vi "CIVI Basic Control Example.vi"() -> ()   [LabVIEW 2026]
panel:
  in  "Frequency Setpoint (Hz)":i32=774000
  out "SCPI Error Code":i32
  in  "Mode Setpint":string="AM"
  out "Operation Complete":string
  out "S Meter (raw)":i32
  out "Mode":string
  out "error out":errorcluster
  out "Frequency (Hz)":i32
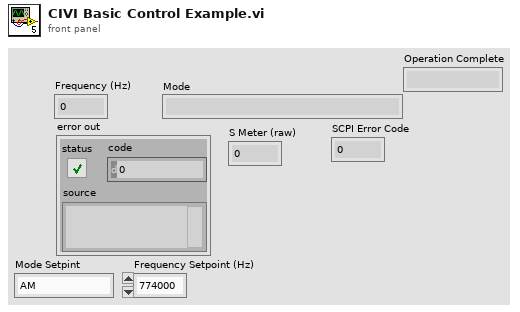
[diagram p1: front panel]
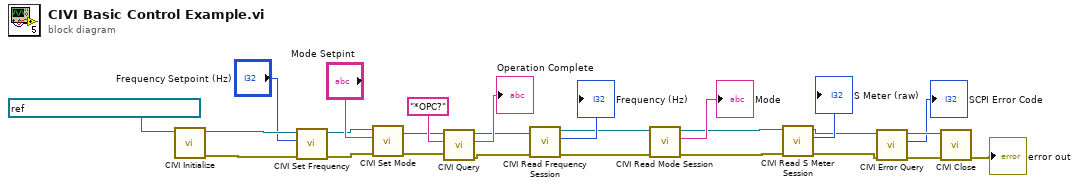
[diagram p0: block diagram]
diagram:
  n1 = call "CIVI Initialize.vi"("VISA Resource Name"=refnum<visa-resource-name> "TCPIP0::127.0.0.1::5025::SOCKET") -> ("error out"=w3:errorcluster, "VISA Session out"=w2:refnum<visa-resource-name>)  [unwired: 9 in]
  n2 = call "CIVI Set Frequency.vi"("error in (no error)"=w3, "Frequency Setpoint (Hz)"="Frequency Setpoint (Hz)", "VISA Refnum in"=w2) -> ("error out"=w4:errorcluster, "VISA Refnum out"=w5:refnum<visa-resource-name>)  [unwired: 7 in]
  n3 = call "CIVI Set Mode.vi"("error in (no error)"=w4, "Mode"="Mode Setpint", "VISA Refnum in"=w5) -> ("error out"=w12:errorcluster, "VISA Refnum out"=w13:refnum<visa-resource-name>)  [unwired: 7 in]
  n4 = call "CIVI Query.vi"("error in"=w12, "write buffer"="*OPC?", "VISA Session in"=w13) -> ("error out"=w14:errorcluster, "read buffer"=→"Operation Complete":string, "VISA Session out"=w15:refnum<visa-resource-name>)  [unwired: 6 in]
  n5 = call "CIVI Read Frequency Session.vi"("error in"=w14, "VISA Session in"=w15) -> ("error out"=w22:errorcluster, "Frequency (Hz)"=→"Frequency (Hz)":i32, "VISA Session out"=w23:refnum<visa-resource-name>)  [unwired: 7 in]
  n6 = call "CIVI Read Mode Session.vi"("error in"=w22, "VISA Session in"=w23) -> ("error out"=w19:errorcluster, "Mode"=→"Mode":string, "VISA Session out"=w20:refnum<visa-resource-name>)  [unwired: 7 in]
  n7 = call "CIVI Read S Meter Session.vi"("error in"=w19, "VISA Session in"=w20) -> ("error out"=w7:errorcluster, "S Meter (raw)"=→"S Meter (raw)":i32, "VISA Session out"=w8:refnum<visa-resource-name>)  [unwired: 7 in]
  n8 = call "CIVI Error Query.vi"("error in"=w7, "VISA Session in"=w8) -> ("error out"=w10:errorcluster, "SCPI Error Code"=→"SCPI Error Code":i32, "VISA Session out"=w9:refnum<visa-resource-name>)  [unwired: 7 in]
  n9 = call "CIVI Close.vi"("error in"=w10, "VISA Session in"=w9) -> ("error out"=→"error out":errorcluster)  [unwired: 9 in]
